vi "Close-database.vi"(8 "error in (no error)":errorcluster caption="错误输入（无错误）", 11 "Database_access 输入":refnum<class "Database_access.lvclass">) -> (0 "error out":errorcluster caption="错误输出", 3 "Database_access 输出":refnum<class "Database_access.lvclass">)   [LabVIEW 2025, in "Database_access.lvclass"]
uses:
  Database_access.lvclass
  Database_access.lvclass/Database_access.ctl
  <vilib>/addons/database/NI_Database_API.lvlib
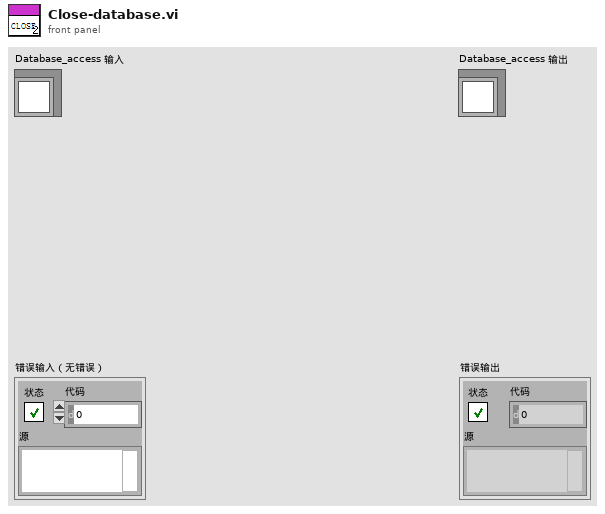
[diagram p1: front panel]
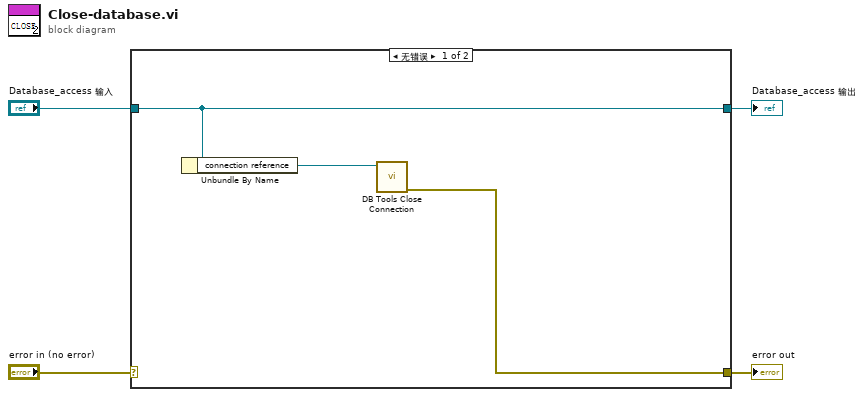
[diagram p0: block diagram]
diagram:
  n1 = case shown="无错误" "error in (no error)" {
    selector: "error in (no error)" -> [_ w9]
    tunnel: [w5 w9] -> w3
    tunnel: [w7 w8] -> w1
    tunnel: "Database_access 输入" -> [w7 w8]
    frame No Error {
      n2 = Unbundle By Name(w7) -> ("connection reference"=w6:refnum<k1>)
      n3 = call <vilib>:"DB Tools Close Connection.vi"("connection reference"=w6) -> ("error out"=w5:errorcluster)  [unwired: 6 in]
    }
    frame Error {
    }
  }
  "error out" <- w3
  "Database_access 输出" <- w1
